vi "WPI_RobotDriveMecanumDrive_Cartesian.vi"(6 "Rotation":dbl, 7 "Gyro Angle":dbl, 8 "error in (no error)":errorcluster, 9 "Y":dbl, 10 "X":dbl, 11 "RobotDriveDevRef":T1={"Motors[]"=[], "Square Inputs"=FALSE, "Max Output"=1.0}) -> (0 "error out":errorcluster, 2 "Motor Values":dbl[](array[numeric]), 3 "RobotDriveDevRef":T1={"Motors[]"=[], "Square Inputs"=FALSE, "Max Output"=1.0})   [LabVIEW 2023]
doc: "Configures the motors for holonomic driving. Holonomic driving allows you to move the robot in any direction without first rotating or maneuvering the robot.\n\nThis VI requires the robot to have either four omni-directional wheels and four motors mounted at 45 degree angles in the four corners of a square frame or to have four mecanum wheels driven by four motors.\n\nThe control input is intended to be connected directly to the X, Y, and Z axes of a joystick. The Y axis is inverted for you.\n\nThis software is licensed. Open the labview\\readme\\WPI Robotics Library Open Source License.txt file for more information."
uses:
  <vilib>/Rock Robotics/WPI/RobotDrive/WPI_RobotDriveDevRef.ctl
  <vilib>/REV Custom Controls/REVSparkRefnum.ctl
  <vilib>/REVLibDriver/REVLibDriver.lvlib
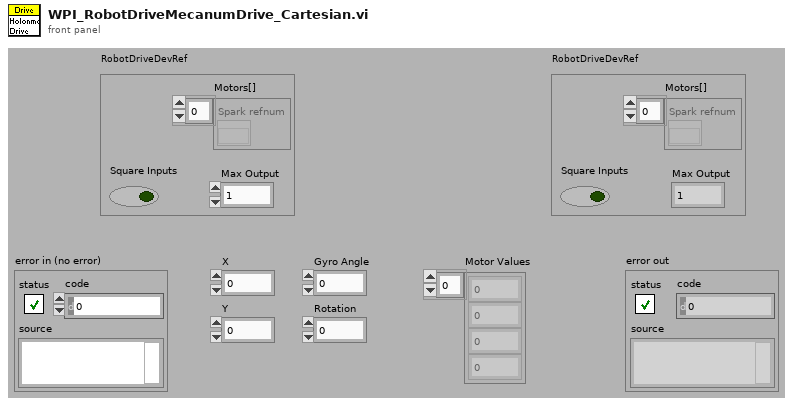
[diagram p1: front panel]
types:
  T1 = typedef "WPI_RobotDriveDevRef.ctl" = cluster{"Motors[]":T2[], "Square Inputs":bool, "Max Output":dbl}
  T2 = typedef "REVLibDriver.lvlib/REVSparkRefnum.ctl" = refnum<k20>
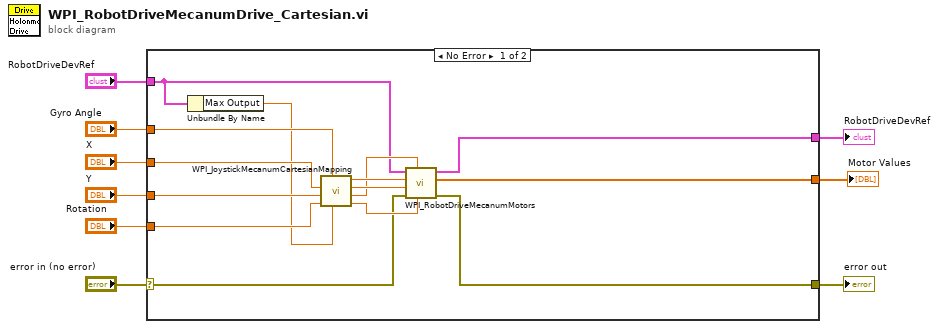
[diagram p0: block diagram]
diagram:
  n1 = case shown="No Error" "error in (no error)" {
    selector: "error in (no error)" -> [w12 w25]
    tunnel: "Y" -> [w22 _]
    tunnel: "X" -> [w21 _]
    tunnel: "RobotDriveDevRef" -> [w11 w24]
    tunnel: [w13 w24] -> w5
    tunnel: [w14 w25] -> w4
    tunnel: "Rotation" -> [w23 _]
    tunnel: "Gyro Angle" -> [w20 _]
    tunnel: [w15 _] -> w1
    frame No Error {
      n2 = Unbundle By Name(w11) -> ("Max Output"=w10:dbl)
      n3 = call <vilib>:"WPI_JoystickMecanumCartesianMapping.vi"("Max Output"=w10, "Gyro Angle"=w20, "Rotation"=w23, "Y"=w22, "X"=w21) -> ("Rear Right"=w19:dbl, "Rear Left"=w16:dbl, "Front Right"=w18:dbl, "Front Left"=w17:dbl)  [unwired: 3 in]
      n4 = call <vilib>:"WPI_RobotDriveMecanumMotors.vi"("Rear Right"=w19, "Rear Left"=w16, "error in"=w12, "Front Right"=w18, "Front Left"=w17, "RobotDriveDevRef in"=w11) -> ("error out"=w14:errorcluster, "Motor Values"=w15:dbl[], "RobotDriveDevRef out"=w13:T1)  [unwired: 3 in]
    }
    frame Error {
    }
  }
  "error out" <- w4
  "RobotDriveDevRef" <- w5
  "Motor Values" <- w1
